vi "PicoScope5000aSetupStreaming.vi"(0 "error in":errorcluster, 1 "Device Info":T2, 2 "handle in":i16, 3 "Acquisition Settings":T3={"Auto Stop"=FALSE, "Desired Sample Interval"=4, "Pre-trigger Samples"=0, "Post-trigger Samples"=1000, "Down-Sample Ratio"=1, "Down-Sample Mode"=0, "Time Units"=2} {"Time Units" items=["Nanoseconds (ns)"=2, "Microseconds (us)"=3, "Milliseconds (ms)"=4, "Seconds (s)"=5]; "Down-Sample Mode" items=["None"=0, "Aggregate"=1, "Decimate"=2, "Average"=4]}, 4 "Buffer and Transfer Settings":T1={"startIndex"=0, "Samples"=1000000, "Down Sample Ratio"=1, "Down-Sample Mode"=0} {"Down-Sample Mode" items=["None"=0, "Aggregate"=1, "Decimate"=2, "Average"=4]; "Down Sample Ratio" step=1; "Samples" format="%_6p"}, 5 "enabled array":i16[](array[numeric]), 10 "Pointers In":u64[][](array[numeric])) -> (11 "Pointer array":u64[][](array[numeric]), 14 "error out":errorcluster, 16 "handle out":i16, 17 "Sample Interval":u32, 19 "sampleIntervalTimeUnits":u32)   [LabVIEW 2010]
doc: "Set up the data buffers and calls RunStreaming to start the device streaming.\nData will be copied from the driver buffers into the corresponding application buffers using the wrapper dll."
uses:
  ps5000a.dll
  ps5000aWrap.dll
panel:
  # "Overview Buffer Size is the size of the temporary buffers used to\nstore data before returning it to the application."
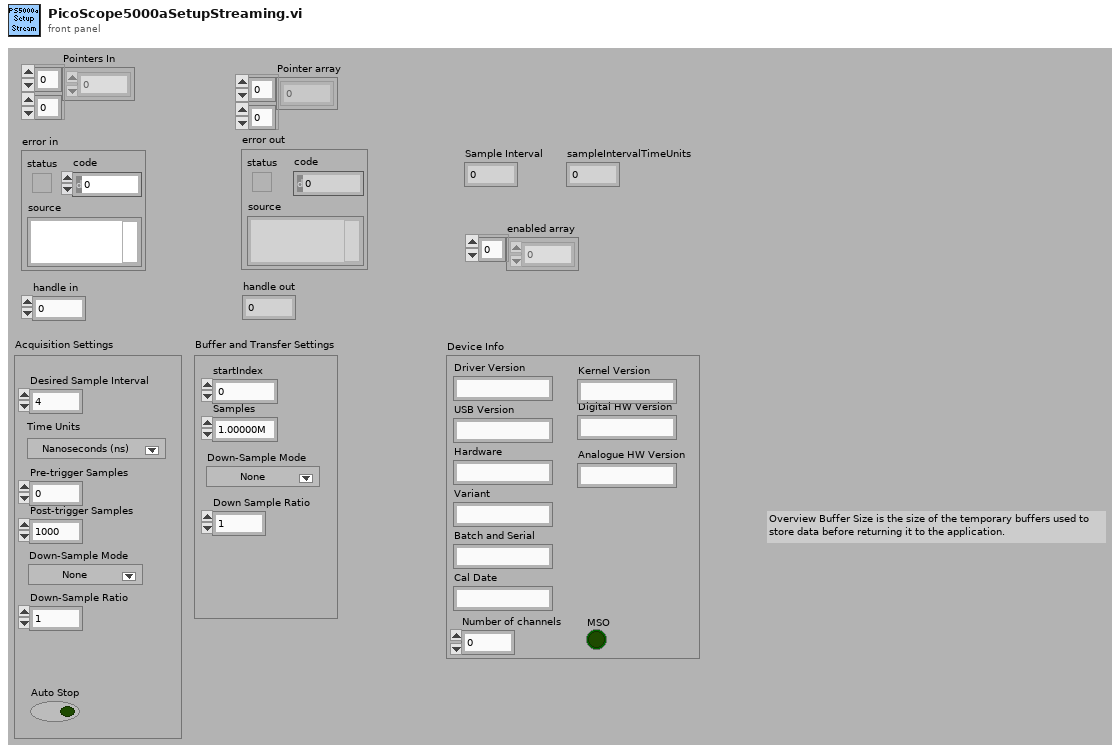
[diagram p1: front panel]
types:
  T1 = cluster{"startIndex":u64, "Samples":u64, "Down Sample Ratio":u64, "Down-Sample Mode":u32}
  T2 = cluster{"Driver Version":string, "USB Version":string, "Hardware":string, "Variant":string, "Batch and Serial":string, "Cal Date":string, "Kernel Version":string, "Digital HW Version":string, "Analogue HW Version":string, "MSO":bool, "Number of channels":i16}
  T3 = cluster{"Auto Stop":bool, "Desired Sample Interval":u32, "Pre-trigger Samples":u32, "Post-trigger Samples":u32, "Down-Sample Ratio":u32, "Down-Sample Mode":i32, "Time Units":u32}
  T4 = cluster{"status":bool, "code":u32, "source":string}
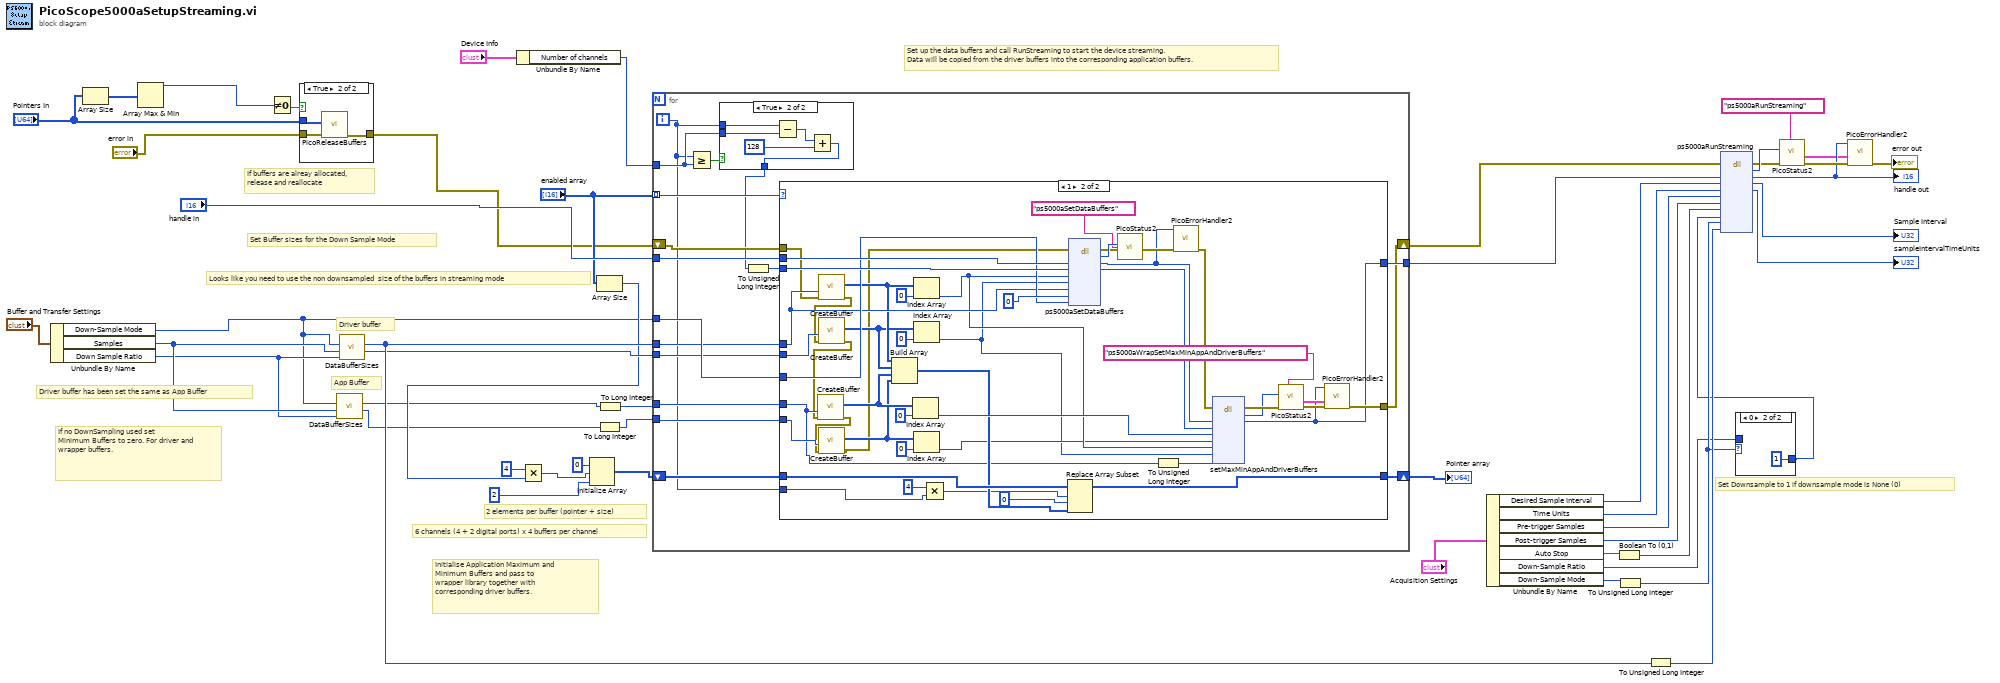
[diagram p0: block diagram]
diagram:
  # "Set up the data buffers and call RunStreaming to start the device streaming.\nData will be copied from the driver buffers into the corresponding application buffers."
  # "Set Downsample to 1 if downsample mode is None (0)"
  # "Looks like you need to use the non downsampled  size of the buffers in streaming mode"
  # "If buffers are alreay allocated,\nrelease and reallocate"
  # "2 elements per buffer (pointer + size)"
  # "6 channels (4 + 2 digital ports) x 4 buffers per channel"
  # "App Buffer"
  # "Driver buffer"
  # "Driver buffer has been set the same as App Buffer"
  # "Set Buffer sizes for the Down Sample Mode"
  # "If no DownSampling used set \nMinimum Buffers to zero. For driver and wrapper buffers."
  # "Initialise Application Maximum and\nMinimum Buffers and pass to \nwrapper library together with corresponding driver buffers."
  n1 = Unbundle By Name("Buffer and Transfer Settings") -> ("Down-Sample Mode"=w10:u32, "Samples"=w33:u64, "Down Sample Ratio"=w32:u64)
  n2 = Array Size(array="Pointers In") -> (size(s)=w13:i32[])
  n3 = Array Max & Min(array=w13) -> (max value=w12:i32)  [unwired: 3 out]
  n4 = Not Equal To 0?(x=w12) -> (x != 0?=w19:bool)
  n5 = case shown="True" w19 {
    tunnel: "Pointers In" -> [_ w52]
    tunnel: "error in" -> [w51 w53]
    tunnel: [w51 w54] -> w16
    frame False {
    }
    frame True {
      n6 = call "PicoReleaseBuffers.vi"("error in (no error)"=w53, "Pointer array"=w52) -> ("error out"=w54:errorcluster)  [unwired: 8 in, 1 out]
    }
  }
  n7 = call "DataBufferSizes.vi"("Down Sample Ratio"=w32, "Number of Samples"=w33, "Down-Sample Mode"=w10) -> ("min Buffer Size"=w3:i32, "Max Buffer Size"=w4:i32)  [unwired: 7 in]
  n8 = call "DataBufferSizes.vi"("Down Sample Ratio"=w32, "Number of Samples"=w33, "Down-Sample Mode"=w10) -> ("min Buffer Size"=w30:i32, "Max Buffer Size"=w31:i32)  [unwired: 7 in]
  n9 = Unbundle By Name("Device Info") -> ("Number of channels"=w2:i16)
  n10 = Array Size(array="enabled array") -> (size(s)=w23:i32)
  n11 = Multiply(x=4, y=w23) -> (x*y=w24:i32)
  n12 = Initialize Array(u64 0 ("element"), w24, 2 ("dimension size")) -> (w14:u64[][])
  n13 = To Long Integer(number=w3) -> (32bit integer=w5:i32)
  n14 = To Long Integer(number=w4) -> (32bit integer=w6:i32)
  n15 = for {
    tunnel: "enabled array" -> [w63] mode=indexing
    tunnel: "handle in" -> [w71]
    tunnel: w10 -> [w70]
    tunnel: w6 -> [w69]
    tunnel: w31 -> [w68]
    tunnel: w30 -> [w67]
    tunnel: w5 -> [w66]
    tunnel: [w64] -> w26
    shift-right: [w62] -> w20
    shift-left: w16 -> [w61]
    shift-right: [w65] -> w29
    shift-left: w14 -> [w60]
    tunnel: w2 -> [w56]
    i -> [w55]
    n16 = Greater Or Equal?(x=w55, y=w56) -> (x >= y?=w58:bool)
    n17 = case shown="True" w58 {
      tunnel: [w72 w76] -> w57
      tunnel: w55 -> [w72 w74]
      tunnel: w56 -> [_ w73]
      frame False {
      }
      frame True {
        n18 = Subtract(x=w74, y=w73) -> (x-y=w75:i32)
        n19 = Add(x=w75, y=128) -> (x+y=w76:i32)
      }
    }
    n20 = To Unsigned Long Integer(number=w57) -> (unsigned 32bit integer=w59:u32)
    n21 = case shown="1" w63 {
      tunnel: w71 -> [w79 w127]
      tunnel: w61 -> [w78 w90]
      tunnel: w59 -> [_ w121]
      tunnel: w69 -> [_ w93]
      tunnel: w68 -> [_ w111]
      tunnel: w67 -> [_ w114]
      tunnel: w66 -> [_ w113]
      tunnel: w70 -> [_ w112]
      tunnel: w60 -> [w80 w105]
      tunnel: [w80 w104] -> w65
      tunnel: w55 -> [_ w101]
      tunnel: [w79 w81] -> w64
      tunnel: [w78 w82] -> w62
      frame 0, Default {
      }
      frame 1 {
        n22 = call "CreateBuffer.vi"("error in (no error)"=w90, "Buffer size"=w111) -> ("error out"=w89:errorcluster, "Pointer and BufferSize"=w109:u64[])  [unwired: 8 in]
        n23 = call "CreateBuffer.vi"("error in (no error)"=w89, "Buffer size"=w114) -> ("error out"=w88:errorcluster, "Pointer and BufferSize"=w108:u64[])  [unwired: 8 in]
        n24 = call "CreateBuffer.vi"("error in (no error)"=w88, "Buffer size"=w93) -> ("error out"=w87:errorcluster, "Pointer and BufferSize"=w107:u64[])  [unwired: 8 in]
        n25 = call "CreateBuffer.vi"("error in (no error)"=w87, "Buffer size"=w113) -> ("error out"=w86:errorcluster, "Pointer and BufferSize"=w106:u64[])  [unwired: 8 in]
        n26 = Build Array(w109, w108, w107, w106) -> (w100:u64[][])
        n27 = Index Array(array=w107, index=0) -> (element=w110:u64)
        n28 = Index Array(array=w109, index=0) -> (element=w103:u64)
        n29 = Index Array(array=w108, index=0) -> (element=w91:u64)
        n30 = Index Array(array=w106, index=0) -> (element=w92:u64)
        n31 = Multiply(x=4, y=w101) -> (x*y=w99:i32)
        n32 = Replace Array Subset(array=w105, new element=w100, index (row)=w99, index (col)=0 ("disabled index (row)")) -> (w104:u64[][])
        n33 = dll-call lib="ps5000a.dll" fn="ps5000aSetDataBuffers" ("ps3000.dll:_ps3000_open_unit@0")(error in=w86, "handle"=w127, "channel"=w121, "bufferMax"=w103, "bufferMin"=w91, "bufferLth"=w111, "segmentIndex"=u32 0, "downSampleRatioMode"=w112) -> (error out=w125:errorcluster, "PICO_STATUS"=w126:u32, "handle"=w95:i16, "channel"=w122:u32)  [unwired: 7 in, 1 out]
        n34 = call "PicoStatus2.vi"("PICO source"="ps5000aSetDataBuffers" ("source"), "Error in"=w125, "PICO STATUS"=w126) -> ("error out"=w97:errorcluster)  [unwired: 5 in, 1 out]
        n35 = To Unsigned Long Integer(number=w93) -> (unsigned 32bit integer=w94:u32)
        n36 = call "PicoErrorHandler2.vi"("error in (no error)"=w97, "handle In"=w95) -> ("error out"=w96:errorcluster)  [unwired: 9 in]
        n37 = dll-call lib="ps5000aWrap.dll" fn="setMaxMinAppAndDriverBuffers"(error in=w96, "handle"=w95, "channel"=w122, "appMaxBuffer"=w110, "appMinBuffer"=w92, "driverMaxBuffer"=w103, "driverMinBuffer"=w91, "bufferLength"=w94) -> (error out=w120:errorcluster, "PICO_STATUS"=w119:u32, "handle"=w81:i16)  [unwired: 8 in, 1 out]
        n38 = call "PicoStatus2.vi"("PICO source"="ps5000aWrapSetMaxMinAppAndDriverBuffers" ("source"), "Error in"=w120, "PICO STATUS"=w119) -> ("error out"=w83:errorcluster, "PICO_STATUS out"=w84:T4)  [unwired: 5 in]
        n39 = call "PicoErrorHandler2.vi"("error in (no error)"=w83, "PICO_STATUS in"=w84, "handle In"=w81) -> ("error out"=w82:errorcluster)  [unwired: 8 in]
      }
    }
  }
  "Pointer array" <- w29
  n40 = Unbundle By Name("Acquisition Settings") -> ("Desired Sample Interval"=w43:u32, "Time Units"=w37:u32, "Pre-trigger Samples"=w42:u32, "Post-trigger Samples"=w41:u32, "Auto Stop"=w40:bool, "Down-Sample Ratio"=w8:u32, "Down-Sample Mode"=w38:i32)
  n41 = Boolean To (0,1)(Boolean=w40) -> (0, 1=w44:i16)
  n42 = To Unsigned Long Integer(number=w38) -> (unsigned 32bit integer=w9:u32)
  n43 = To Unsigned Long Integer(number=w31) -> (unsigned 32bit integer=w11:u32)
  n44 = case shown="0" w9 {
    tunnel: [w128 u32 1 ("Down-Sample Ratio")] -> w7
    tunnel: w8 -> [w128 _]
    frame Default {
    }
    frame 0 {
    }
  }
  n45 = dll-call lib="ps5000a.dll" fn="ps5000aRunStreaming" ("ps5000a.dll:_ps3000_open_unit@0")(error in=w20, "handle"=w26, "sampleInterval"=w43, "sampleIntervalTimeUnits"=w37, "maxPreTriggerSamples"=w42, "maxPostTriggerSamples"=w41, "autoStop"=w44, "downSampleRatio"=w7, "downSampleRatioMode"=w9, "overviewBufferSize"=w11) -> (error out=w48:errorcluster, "PICO_STATUS"=w49:u32, "handle"=w15:i16, "sampleInterval"=→"Sample Interval":u32, "sampleIntervalTimeUnits"=→"sampleIntervalTimeUnits":u32)  [unwired: 8 in, 1 out]
  "handle out" <- w15
  n46 = call "PicoStatus2.vi"("PICO source"="ps5000aRunStreaming" ("source"), "Error in"=w48, "PICO STATUS"=w49) -> ("error out"=w46:errorcluster, "PICO_STATUS out"=w1:T4)  [unwired: 5 in]
  n47 = call "PicoErrorHandler2.vi"("error in (no error)"=w46, "PICO_STATUS in"=w1, "handle In"=w15) -> ("error out"=→"error out":errorcluster)  [unwired: 8 in]
